vi "Right Read Insertion_MS_IDX.vi"(6 "Total assembly C":T2 {"Assembly Ratio 2" format="%#_3g"; "Assembly Ratio" format="%#_3g"}, 8 "error in":errorcluster, 9 "Signal Tag":string[](array[string]), 10 "SOC cluster":T1, 11 "Signal Profile Table":string[][](table) caption="Singla Profile Table") -> (0 "error out":errorcluster, 1 "ASM C":T4, 2 "Signal Number Histogram":cluster{"配列 2":i32[], "配列 5":dbl[]}[](graph), 3 "BS Table":string[][](table), 4 "LSP Table":string[][](table), 5 "LSS Tag":T3)   [LabVIEW 2018]
panel:
  out "appended array":string[][](array[string])
  out "Selected L#":i32[](array[numeric])
  out "Sample Sequence":string
  out "Selected S IDX":i32[](array[numeric])
  out "サイズ":i32
  out "L Signal Tag A":string[](array[string])
  out "Long Signal#":i32
  out "AR#":i32[](array[numeric])
  out "RR#":i32[](array[numeric])
  out "assembly C":T5
  out "Long Assembly":bool[][](array[boolean])
  out "Right Read MIN":i32=5
  out "Signal Tag A":string[](array[string])
  out "平均 RR Read N":dbl format="%#_4g"
  out "RR シグナル集計":dbl[][](array[numeric])
  out "平均 Read N":dbl format="%#_4g"
  out "シグナル集計":dbl[][](array[numeric])
  out "All assembly":bool[][](array[boolean])
  out "Cutted Sample Sequence":string
  out "Signal#":i32
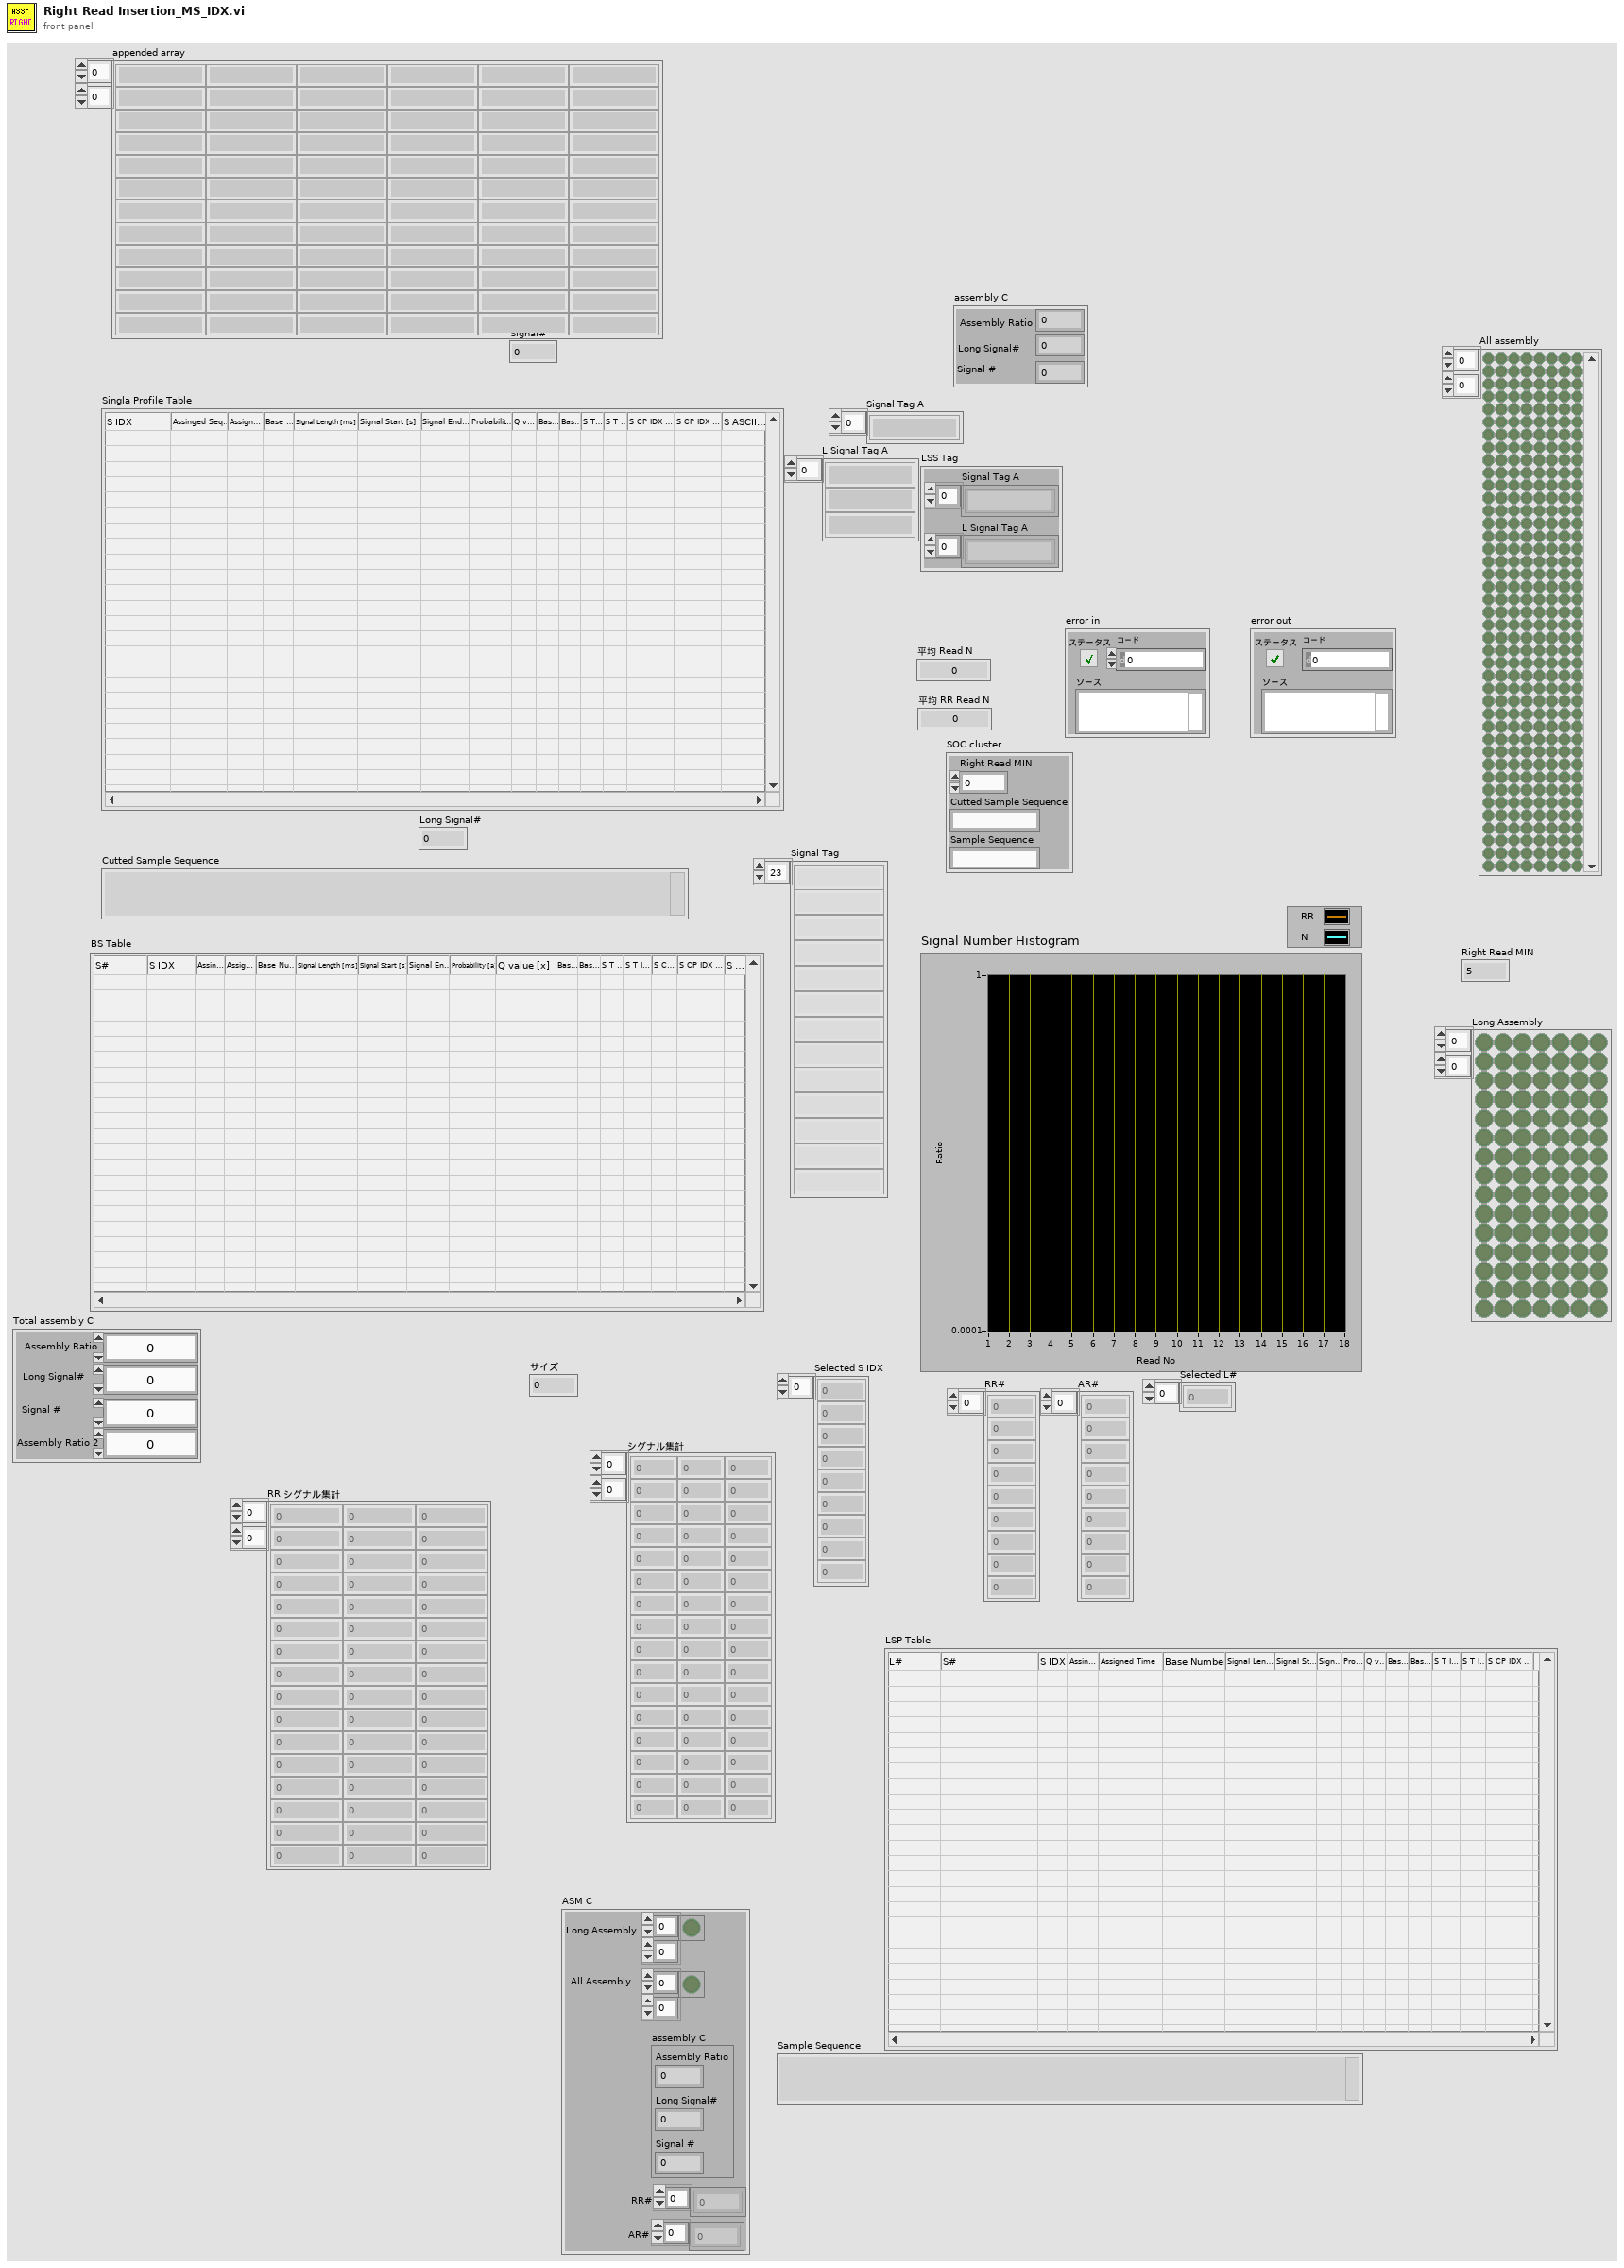
[diagram p1: front panel]
types:
  T1 = cluster{"Right Read MIN":i32, "Cutted Sample Sequence":string, "Sample Sequence":string}
  T2 = cluster{"Assembly Ratio":dbl, "Long Signal#":i32, "Signal #":i32, "Assembly Ratio 2":dbl}
  T3 = cluster{"Signal Tag A":string[], "L Signal Tag A":string[]}
  T4 = cluster{"Long Assembly":bool[][], "All Assembly":bool[][], "assembly C":cluster{"Assembly Ratio":dbl, "Long Signal#":i32, "Signal #":i32}, "RR#":i32[], "AR#":i32[]}
  T5 = cluster{"Assembly Ratio":dbl, "Long Signal#":i32, "Signal #":i32}
  T6 = cluster{"Read Seq":string, "Read No":i32, "Mx Right Read":string, "Mx No":i32, "Dir":enum16{"5’→3'", "3'→5'"}, "Front Seq":string, "Seq":string, "Later Seq":string, bool, "Seq SNo":i32, "Seq ENo":i32}
  T7 = cluster{"Long Assembly":bool[][], bool[][], "assembly C":cluster{"Assembly Ratio":dbl, "Long Signal#":i32, "Signal #":i32}, i32[], "Value":i32[]}
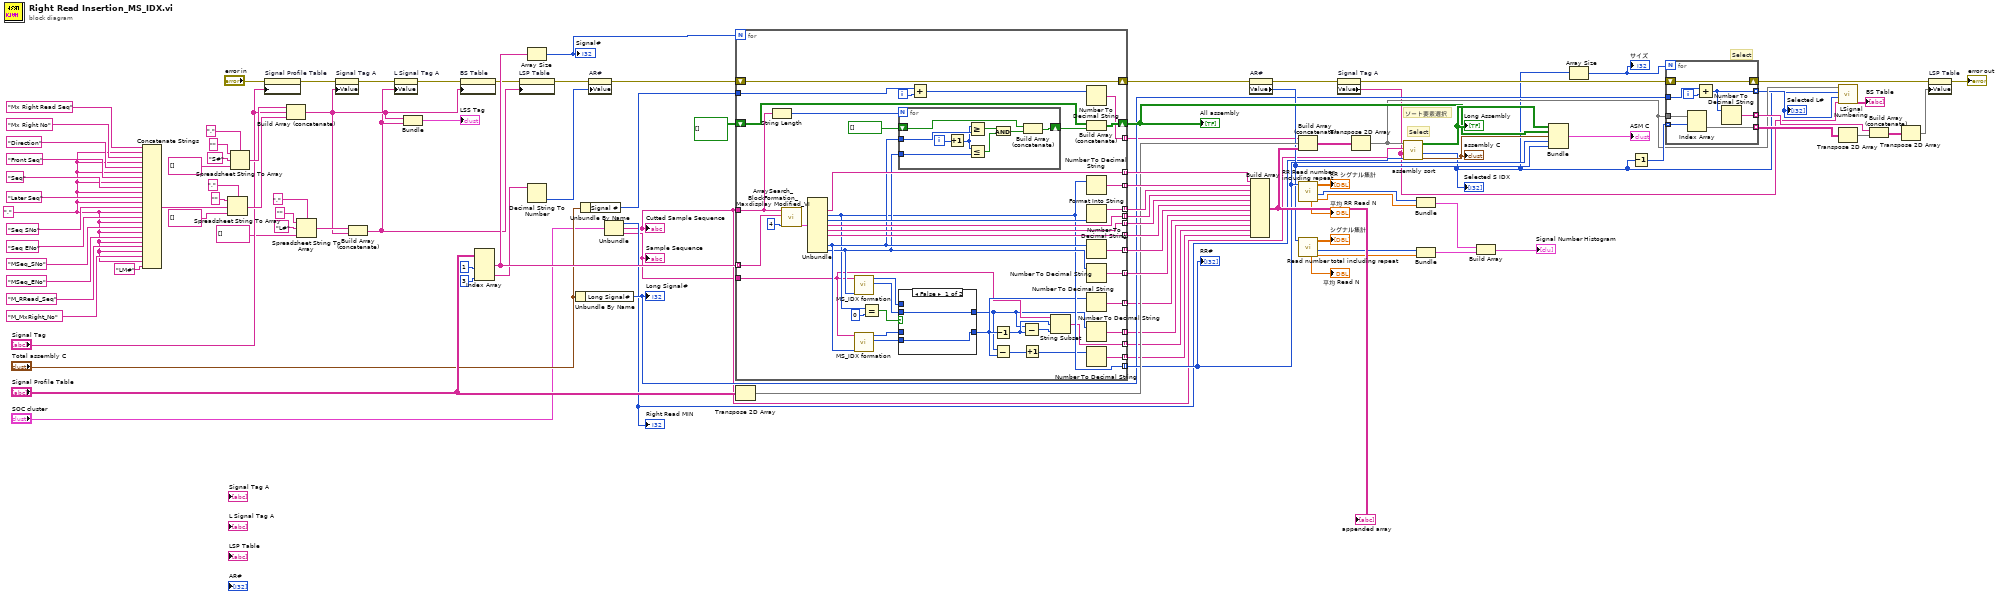
[diagram p0: block diagram]
diagram:
  w6 = "," ("デリミタ（タブ）")
  # "Select"
  # "Select"
  # "ソート要素選択"
  n1 = Concatenate Strings("Mx Right Read Seq" ("文字列"), w6, "Mx Right No" ("文字列"), w6, "Direction" ("文字列"), w6, "Front Seq" ("文字列"), w6, "Seq" ("文字列"), w6, "Later Seq" ("文字列"), w6, "Seq SNo" ("文字列"), w6, "Seq ENo" ("文字列"), w6, "MSeq_SNo" ("文字列"), w6, "MSeq_ENo" ("文字列"), w6, "M_RRead_Seq" ("文字列"), w6, "M_MxRight_No" ("文字列"), w6, "LM#" ("文字列")) -> (w74:string)
  n2 = Spreadsheet String To Array(delimiter (Tab)="," ("デリミタ（タブ）"), format string="" ("形式文字列"), spreadsheet string=w74, array type (2D Dbl)=string[] [] ("行ヘッダ文字列[]")) -> (array=w41:string[])
  n3 = Spreadsheet String To Array(delimiter (Tab)="," ("デリミタ（タブ）"), format string="" ("形式文字列"), spreadsheet string="S#" ("文字列"), array type (2D Dbl)=string[] [] ("行ヘッダ文字列[]")) -> (array=w47:string[])
  n4 = property on="Signal Profile Table" class="Tbl (strict)"(error in="error in", "Column Headers[]"="Signal Tag") -> (error out=w29:errorcluster)  [unwired: 1 in, 1 out]
  n5 = Build Array (concatenate)(w47, "Signal Tag", w41) -> (w30:string[])
  n6 = Spreadsheet String To Array(delimiter (Tab)="," ("デリミタ（タブ）"), format string="" ("形式文字列"), spreadsheet string="L#" ("文字列"), array type (2D Dbl)=string[] [] ("行ヘッダ文字列[]")) -> (array=w33:string[])
  n7 = property on="Signal Tag A" class="Arr (strict)"(error in=w29, "Value"=w30) -> (error out=w28:errorcluster)  [unwired: 1 in, 1 out]
  n8 = Build Array (concatenate)(w33, w30) -> (w26:string[])
  n9 = property on="L Signal Tag A" class="Arr (strict)"(error in=w28, "Value"=w26) -> (error out=w27:errorcluster)  [unwired: 1 in, 1 out]
  n10 = Bundle(w30, w26) -> (→"LSS Tag":cluster{string[], string[]})  [unwired: 1 in]
  n11 = property on="BS Table" class="Tbl (strict)"(error in=w27, "Column Headers[]"=w30) -> (error out=w39:errorcluster)  [unwired: 1 in, 1 out]
  n12 = Index Array(array="Signal Profile Table", index (col) #1=1 ("無効な指標 （列）"), index (col) #2=3 ("指標 （列）")) -> (element #1=w104:string[], element #2=w90:string[])  [unwired: 2 in]
  n13 = property on="LSP Table" class="Tbl (strict)"(error in=w39, "Column Headers[]"=w26) -> (error out=w38:errorcluster)  [unwired: 1 in, 1 out]
  n14 = Array Size(array=w104) -> (size(s)=w65:i32)
  "Signal#" <- w65
  n15 = Decimal String To Number(string=w90) -> (number=w56:i32[])  [unwired: 2 in, 1 out]
  n16 = Unbundle By Name("Total assembly C") -> ("Long Signal#"=w45:i32)
  "Long Signal#" <- w45
  n17 = Unbundle By Name("Total assembly C") -> ("Signal #"=w42:i32)
  n18 = property on="AR#" class="Arr (strict)"(error in=w38, "Value"=w56) -> (error out=w55:errorcluster)  [unwired: 1 in, 1 out]
  n19 = Unbundle("SOC cluster") -> ("Right Read MIN"=w21:i32, "Cutted Sample Sequence"=w20:string, "Sample Sequence"=w19:string)
  "Cutted Sample Sequence" <- w20
  "Right Read MIN" <- w21
  "Sample Sequence" <- w19
  n20 = for {
    N: w65 -> [_]
    tunnel: w104 -> [w133] mode=indexing
    tunnel: w20 -> [w134]
    tunnel: [w148] -> w103 mode=indexing
    tunnel: [w147] -> w102 mode=indexing
    tunnel: [w145] -> w101 mode=indexing
    tunnel: [w144] -> w100 mode=indexing
    tunnel: [w143] -> w99 mode=indexing
    tunnel: [w142] -> w98 mode=indexing
    tunnel: [w141] -> w97 mode=indexing
    tunnel: [w140] -> w96 mode=indexing
    shift-right: [w137] -> w63
    shift-left: bool[][] [] -> [w136]
    tunnel: [w118] -> w59 mode=indexing
    shift-right: [w130] -> w54
    shift-left: w55 -> [w130]
    tunnel: w42 -> [w129]
    tunnel: [w126] -> w32 mode=indexing
    tunnel: w19 -> [w108]
    tunnel: [w116] -> w16 mode=indexing
    tunnel: [w115] -> w15 mode=indexing
    tunnel: [w112] -> w13 mode=indexing
    tunnel: [w106] -> w14 mode=indexing
    i -> [w128]
    n21 = String Length(string=w134) -> (length=w139:i32)
    n22 = call "ArraySearch_BlockFormation_Maxdisplay Modified_VI.vi"("RR number"=4, "読み取り配列"=w133, "Cutted Sample Sequence"=w134) -> ("出力クラスタ 2"=w131:T6)  [unwired: 8 out]
    n23 = Unbundle(w131) -> ("Mx Right Read"=w148:string, "Mx No"=w118:i32, "Dir"=w146:enum16{"5’→3'", "3'→5'"}, "Front Seq"=w144:string, "Seq"=w143:string, "Later Seq"=w142:string, "Seq SNo"=w125:i32, "Seq ENo"=w124:i32)  [unwired: 3 out]
    n24 = call "MS_IDX formation.vi"("AS_ISX"=w124, "Sample sequnce"=w108) -> ("MS_IXD3"=w119:i32, "MS_IXD5"=w121:i32)  [unwired: 7 in, 1 out]
    n25 = call "MS_IDX formation.vi"("AS_ISX"=w125, "Sample sequnce"=w108) -> ("MS_IXD3"=w120:i32, "MS_IXD5"=w122:i32)  [unwired: 7 in, 1 out]
    n26 = Equal?(x=w118, y=0) -> (x = y?=w123:bool)
    n27 = for {
      N: w139 -> [_]
      tunnel: w125 -> [w154]
      tunnel: w124 -> [w156]
      shift-right: [w161] -> w138
      shift-left: bool[] [] -> [w160]
      i -> [w155]
      n28 = Increment(x=w155) -> (x+1=w153:i32)
      n29 = Greater Or Equal?(x=w153, y=w154) -> (x >= y?=w159:bool)
      n30 = Less Or Equal?(x=w153, y=w156) -> (x <= y?=w157:bool)
      n31 = And(x=w159, y=w157) -> (x .and. y?=w158:bool)
      n32 = Build Array (concatenate)(w160, w158) -> (w161:bool[])
    }
    n33 = case shown="False" w123 {
      tunnel: w122 -> [_ w152]
      tunnel: w121 -> [_ w151]
      tunnel: w120 -> [w150 _]
      tunnel: w119 -> [w149 _]
      tunnel: [w150 w152] -> w109
      tunnel: [w149 w151] -> w107
      frame False {
      }
      frame True {
      }
    }
    n34 = Add(x=w129, y=w128) -> (x+y=w127:i32)
    n35 = Decrement(x=w109) -> (x-1=w111:i32)
    n36 = Subtract(x=w107, y=w109) -> (x-y=w114:i32)
    n37 = Subtract(x=w107, y=w111) -> (x-y=w110:i32)
    n38 = Increment(x=w114) -> (x+1=w113:i32)
    n39 = String Subset(string=w108, offset (0)=w111, length (rest)=w110) -> (substring=w106:string)
    n40 = Number To Decimal String(number=w127) -> (decimal integer string=w126:string)  [unwired: 1 in]
    n41 = Build Array (concatenate)(w136, w138) -> (w137:bool[][])
    n42 = Number To Decimal String(number=w118) -> (decimal integer string=w147:string)  [unwired: 1 in]
    n43 = Format Into String(w146) -> (resulting string=w145:string)  [unwired: 3 in, 1 out]
    n44 = Number To Decimal String(number=w125) -> (decimal integer string=w141:string)  [unwired: 1 in]
    n45 = Number To Decimal String(number=w124) -> (decimal integer string=w140:string)  [unwired: 1 in]
    n46 = Number To Decimal String(number=w109) -> (decimal integer string=w116:string)  [unwired: 1 in]
    n47 = Number To Decimal String(number=w107) -> (decimal integer string=w115:string)  [unwired: 1 in]
    n48 = Number To Decimal String(number=w113) -> (decimal integer string=w112:string)  [unwired: 1 in]
  }
  "All assembly" <- w63
  "RR#" <- w59
  n49 = Transpose 2D Array(2D array="Signal Profile Table") -> (transposed array=w94:string[][])
  n50 = property on="AR#" class="Arr (strict)"(error in=w54) -> (error out=w52:errorcluster, "Value"=w53:i32[])  [unwired: 1 in, 1 out]
  n51 = Build Array(w103, w102, w101, w100, w99, w98, w97, w96, w16, w15, w14, w13) -> (w93:string[][])
  "appended array" <- w93
  n52 = Build Array (concatenate)(w32, w94, w93) -> (w66:string[][])
  n53 = call "RR Read number including repeat.vi"("RR Read No"=w59) -> ("RR %"=w85:dbl[], "RR N#"=w84:i32[], "シグナル集計"=→"RR シグナル集計":dbl[][], "Average Read N"=→"平均 RR Read N":dbl)  [unwired: 3 in, 4 out]
  n54 = call "Read number total including repeat.vi"("Read No"=w53) -> ("AR %"=w82:dbl[], "AR N#"=w83:i32[], "シグナル集計"=→"シグナル集計":dbl[][], "平均 Read N"=→"平均 Read N":dbl)  [unwired: 2 in, 5 out]
  n55 = property on="Signal Tag A" class="Arr (strict)"(error in=w52) -> (error out=w51:errorcluster, "Value"=w9:string[])  [unwired: 1 in, 1 out]
  n56 = Transpose 2D Array(2D array=w66) -> (transposed array=w10:string[][])
  n57 = call "assembly sort.vi"("Right Read MIN"=w21, "Signal Tag A"=w9, "連続排除配列"=w20, "Signal Profile Table A"=w10) -> ("assembly C"=w62:T5, "Selected S IDX"=w7:i32[], "Long Assembly"=w64:bool[][])  [unwired: 3 in, 2 out]
  "Long Assembly" <- w64
  "assembly C" <- w62
  "Selected S IDX" <- w7
  n58 = Bundle("RR N#"=w84, "RR %"=w85) -> (w81:cluster{"RR N#":i32[], "RR %":dbl[]})  [unwired: 1 in]
  n59 = Bundle("AR N#"=w83, "AR %"=w82) -> (w80:cluster{"AR N#":i32[], "AR %":dbl[]})  [unwired: 1 in]
  n60 = Build Array(w81, w80) -> (→"Signal Number Histogram":cluster{"AR N#":i32[], "AR %":dbl[]}[])
  n61 = Bundle("Long Assembly"=w64, w63, "assembly C"=w62, w59, "Value"=w53) -> (→"ASM C":T7)  [unwired: 1 in]
  n62 = Array Size(array=w7) -> (size(s)=w61:i32)
  "サイズ" <- w61
  n63 = Decrement(x=w7) -> (x-1=w60:i32[])
  n64 = for {
    N: w61 -> [_]
    tunnel: w10 -> [w169]
    tunnel: w60 -> [w168] mode=indexing
    tunnel: [w167] -> w43 mode=indexing
    shift-right: [w166] -> w2
    shift-left: w51 -> [w166]
    tunnel: w45 -> [w165]
    tunnel: [w163] -> w44 mode=indexing
    tunnel: [w162] -> w8 mode=indexing
    i -> [w164]
    n65 = Index Array(array=w169, index (row)=w168) -> (element=w167:string[])  [unwired: 1 in]
    n66 = Add(x=w165, y=w164) -> (x+y=w162:i32)
    n67 = Number To Decimal String(number=w162) -> (decimal integer string=w163:string)  [unwired: 1 in]
  }
  "Selected L#" <- w8
  n68 = call "LSignal Numbering.vi"("Signal Tag A"=w9, "Selected L#"=w8, "Selected S IDX"=w7, "Signal Profile Table A"=w10) -> ("BS Table"=→"BS Table":string[][])  [unwired: 6 in, 1 out]
  n69 = Transpose 2D Array(2D array=w43) -> (transposed array=w24:string[][])
  n70 = Build Array (concatenate)(w44, w24) -> (w25:string[][])
  n71 = Transpose 2D Array(2D array=w25) -> (transposed array=w3:string[][])
  n72 = property on="LSP Table" class="Tbl (strict)"(error in=w2, "Value"=w3) -> (error out=→"error out":errorcluster)  [unwired: 1 in, 1 out]
